vi "Run_Protocol_Tests_CLI.vi"(11 "Command Line Arguments":string[](array[string])) -> (2 "Output":string, 3 "Exit Code":i32)   [LabVIEW 2020, in "MCP Server tests.lvlib"]
doc: "Runs the protocol tester tools\\test\\Test-McpServer.ps1 against a test MCP server and passes the result to LabVIEW CLI. The server is started with Start.vi on port 36987 at /mcp/server and gets the Caraya suite's fixture resources, prompt and tool, so tools, prompts and resources are all declared. The tester runs through System Exec and its standard output and standard error are written to results\\protocol-report.txt next to this VI, overwriting an older report. The server is always stopped with Stop.vi, also when the tester or an earlier step failed.\n\nExit Code is 0 when the tester returned 0 (no failed required check) and no error occurred, and 1 otherwise. Output is a one-line summary. Errors are cleared at the end so the VI always returns."
uses:
  dfe142dc-6e41-4d89-b458-133232547ee5.vi
  src/MCP Server/MCP Server.lvlib
  MCP Server tests.lvlib
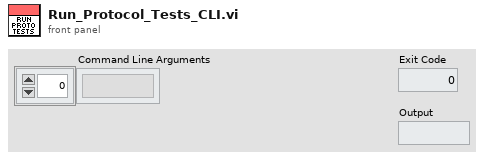
[diagram p1: front panel]
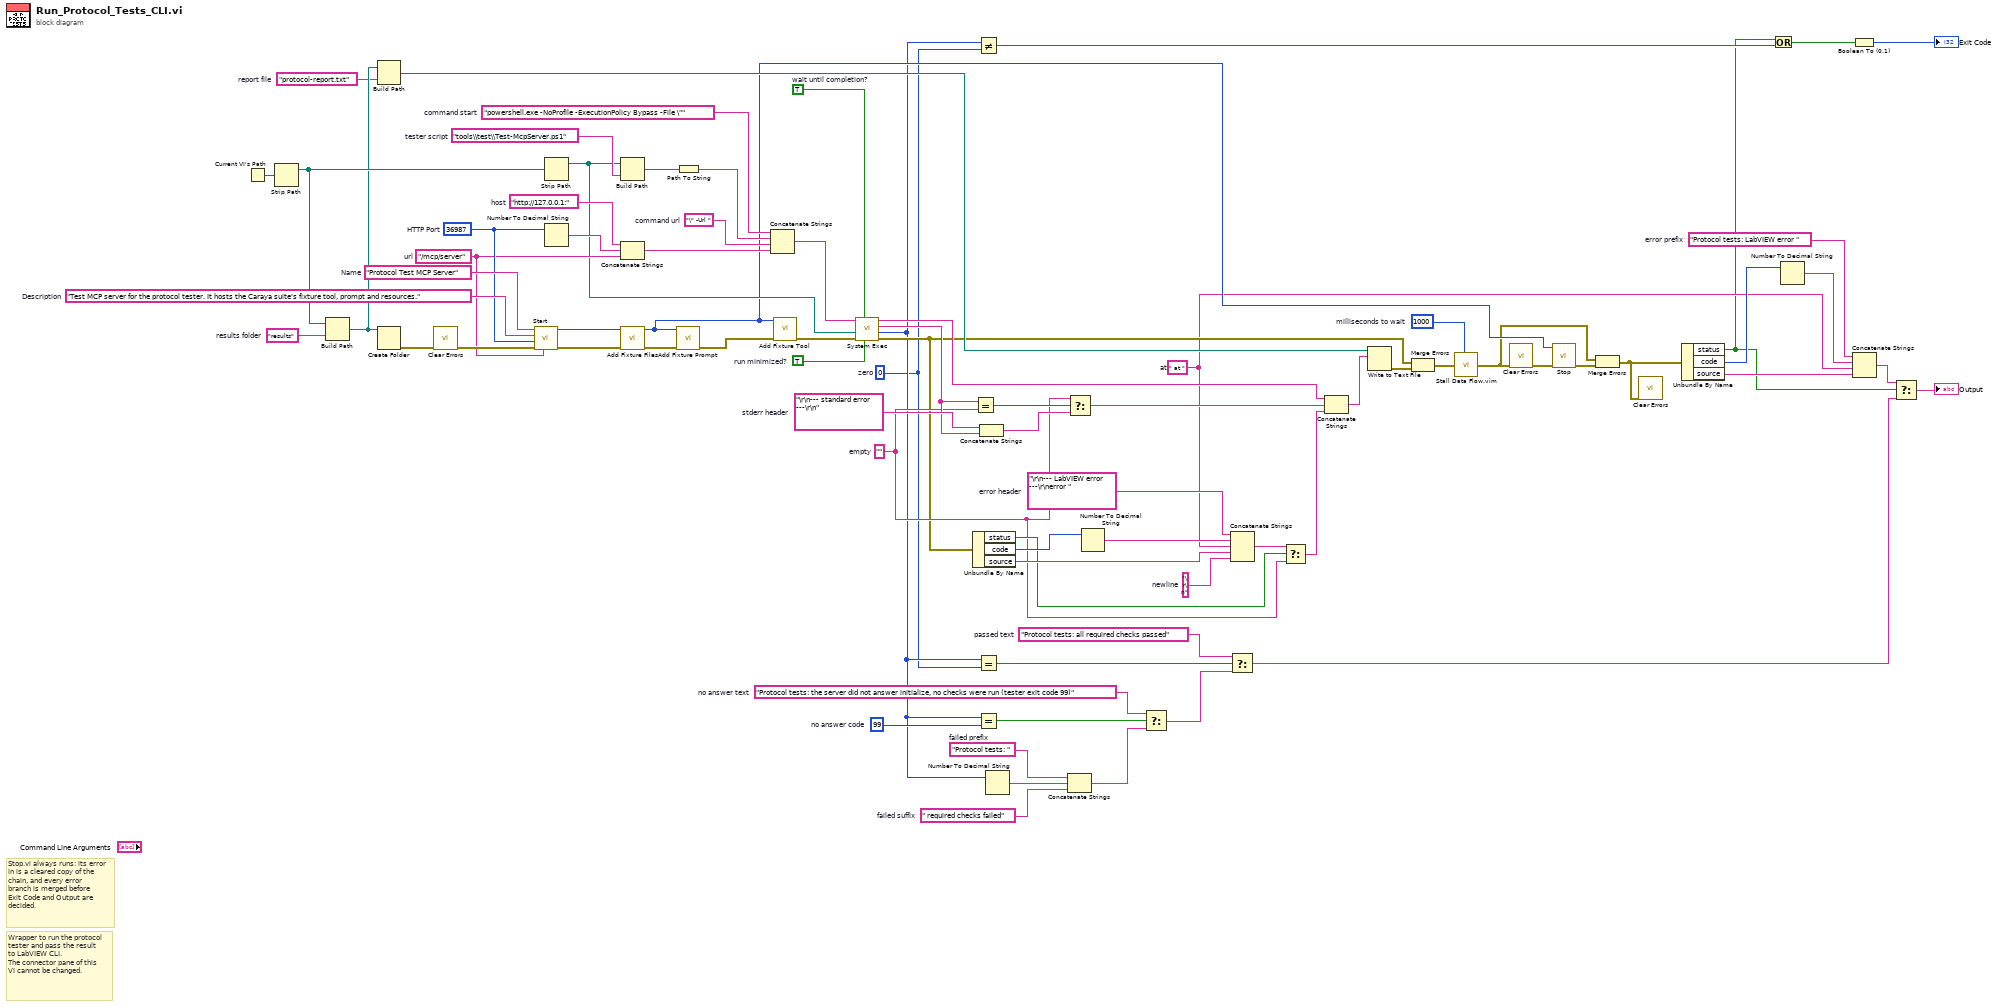
[diagram p0: block diagram]
diagram:
  w19 = "Protocol tests: LabVIEW error "  # error prefix
  w21 = " required checks failed"  # failed suffix
  w23 = "Protocol tests: "  # failed prefix
  w12 = "Protocol tests: the server did not answer initialize, no checks were run (tester exit code 99)"  # no answer text
  w9 = "Protocol tests: all required checks passed"  # passed text
  w15 = 99  # no answer code
  w13 = 0  # zero
  w30 = u32 1000  # milliseconds to wait
  w42 = "\r\n"  # newline
  w17 = " at "  # at
  w45 = "\r\n--- LabVIEW error ---\r\nerror "  # error header
  w50 = "\r\n--- standard error ---\r\n"  # stderr header
  w39 = ""  # empty
  w51 = TRUE  # run minimized?
  w52 = TRUE  # wait until completion?
  w57 = "\" -Url "  # command url
  w59 = "powershell.exe -NoProfile -ExecutionPolicy Bypass -File \""  # command start
  w62 = "http://127.0.0.1:"  # host
  w60 = "/mcp/server"  # url
  w63 = u16 36987  # HTTP Port
  w69 = "Test MCP server for the protocol tester. It hosts the Caraya suite's fixture tool, prompt and resources."  # Description
  w70 = "Protocol Test MCP Server"  # Name
  w73 = "tools\\test\\Test-McpServer.ps1"  # tester script
  w74 = "protocol-report.txt"  # report file
  w76 = "results"  # results folder
  # "Stop.vi always runs: its error in is a cleared copy of the chain, and every error branch is merged before Exit Code and Output are decided."
  # "Wrapper to run the protocol tester and pass the result to LabVIEW CLI.\nThe connector pane of this VI cannot be changed."
  n1 = Current VI's Path() -> (path=w78:path)
  n2 = Strip Path(path=w78) -> (stripped path=w77:path)  [unwired: 1 out]
  n3 = Build Path(base path=w77, name or relative path=w76) -> (appended path=w75:path)
  n4 = Build Path(base path=w75, name or relative path=w74) -> (appended path=w35:path)
  n5 = Create Folder(path (use dialog)=w75) -> (error out=w71:errorcluster)  [unwired: 2 in, 2 out]
  n6 = call <vilib>:"Clear Errors.vi"("error in (no error)"=w71) -> ("error out"=w68:errorcluster)  [unwired: 5 in, 1 out]
  n7 = call "Start.vi"("url (\"/mcp/server\")"=w60, "error in (no error)"=w68, "HTTP Port (36987)"=w63, "Description"=w69, "Name"=w70) -> ("error out"=w66:errorcluster, "server id out"=w67:i32)  [unwired: 4 in, 1 out]
  n8 = Strip Path(path=w77) -> (stripped path=w54:path)  [unwired: 1 out]
  n9 = Number To Decimal String(number=w63) -> (decimal integer string=w61:string)  [unwired: 1 in]
  n10 = Build Path(base path=w54, name or relative path=w73) -> (appended path=w72:path)
  n11 = Concatenate Strings(w62, w61, w60) -> (w56:string)
  n12 = call "Add Fixture Files.vi"("error in (no error)"=w66, "server id"=w67) -> ("error out"=w65:errorcluster, "server id out"=w29:i32)  [unwired: 8 in]
  n13 = call "Add Fixture Prompt.vi"("error in (no error)"=w65, "server id"=w29) -> ("error out"=w64:errorcluster)  [unwired: 8 in, 1 out]
  n14 = Path To String(path=w72) -> (string=w58:string)
  n15 = Concatenate Strings(w59, w58, w57, w56) -> (w55:string)
  n16 = call "Add Fixture Tool.vi"("error in (no error)"=w64, "server id"=w29) -> ("error out"=w53:errorcluster)  [unwired: 8 in, 1 out]
  n17 = call <vilib>:"System Exec.vi"("run minimized? (F)"=w51, "wait until completion? (T)"=w52, "error in (no error)"=w53, "working directory"=w54, "command line"=w55) -> ("error out"=w33:errorcluster, "return code"=w14:i32, "standard error"=w49:string, "standard output"=w38:string)  [unwired: 3 in]
  n18 = Unbundle By Name(w33) -> ("status"=w40:bool, "code"=w46:i32, "source"=w43:string)
  n19 = Equal?(x=w49, y=w39) -> (x = y?=w48:bool)
  n20 = Not Equal?(x=w14, y=w13) -> (x != y?=w25:bool)
  n21 = Equal?(x=w14, y=w13) -> (x = y?=w8:bool)
  n22 = Equal?(x=w14, y=w15) -> (x = y?=w11:bool)
  n23 = Concatenate Strings(w50, w49) -> (w47:string)
  n24 = Number To Decimal String(number=w14) -> (decimal integer string=w22:string)  [unwired: 1 in]
  n25 = Concatenate Strings(w23, w22, w21) -> (w10:string)
  n26 = Select(t=w39, s=w48, f=w47) -> (s? t:f=w37:string)
  n27 = Number To Decimal String(number=w46) -> (decimal integer string=w44:string)  [unwired: 1 in]
  n28 = Select(t=w12, s=w11, f=w10) -> (s? t:f=w7:string)
  n29 = Concatenate Strings(w45, w44, w17, w43, w42) -> (w41:string)
  n30 = Select(t=w9, s=w8, f=w7) -> (s? t:f=w4:string)
  n31 = Select(t=w41, s=w40, f=w39) -> (s? t:f=w36:string)
  n32 = Concatenate Strings(w38, w37, w36) -> (w34:string)
  n33 = Write to Text File(file (use dialog)=w35, text=w34) -> (error out=w32:errorcluster)  [unwired: 2 in, 2 out]
  n34 = Merge Errors(w33, w32) -> (w31:errorcluster)
  n35 = call "Stall Data Flow.vim"("value in"=w31, "milliseconds to wait"=w30) -> ("value out"=w27:errorcluster)  [unwired: 1 out]
  n36 = call <vilib>:"Clear Errors.vi"("error in (no error)"=w27) -> ("error out"=w28:errorcluster)  [unwired: 5 in, 1 out]
  n37 = call "Stop.vi"("error in (no error)"=w28, "id"=w29) -> ("error out"=w26:errorcluster)  [unwired: 9 in]
  n38 = Merge Errors(w27, w26) -> (w3:errorcluster)
  n39 = call <vilib>:"Clear Errors.vi"("error in (no error)"=w3) -> ()  [unwired: 5 in, 2 out]
  n40 = Unbundle By Name(w3) -> ("status"=w5:bool, "code"=w20:i32, "source"=w16:string)
  n41 = Or(x=w5, y=w25) -> (x .or. y?=w24:bool)
  n42 = Number To Decimal String(number=w20) -> (decimal integer string=w18:string)  [unwired: 1 in]
  n43 = Boolean To (0,1)(Boolean=w24) -> (0, 1=→"Exit Code":i16)
  n44 = Concatenate Strings(w19, w18, w17, w16) -> (w6:string)
  n45 = Select(t=w6, s=w5, f=w4) -> (s? t:f=→"Output":string)
